vi "2006_FireAtSpecificTimeOnSpecificWeekdays.vi"(8 "error in (no error)":errorcluster) -> (0 "error out":errorcluster)   [LabVIEW 2013]
uses:
  source/Cron.Jenkins/Cron.Jenkins.lvclass/Cron.Jenkins.ctl
  source/Cron.Jenkins/Write Job Name.vi
  <vilib>/addons/_JKI Toolkits/Caraya/classes/Assert/Assert True.vi
  source/Cron/Create Cron Expression.vi
  source/Cron/Compute Next Cron.vi
  source/Cron.Jenkins/Cron.Jenkins.lvclass
  <vilib>/addons/_JKI Toolkits/Caraya/classes/Test/Test.lvclass
  <vilib>/addons/_JKI Toolkits/Caraya/classes/Assert/Assert.lvclass
  source/openCron.lvlib
panel:
  out "after weekend":timestamp
  out "Occurences":timestamp[](array[timestamp])
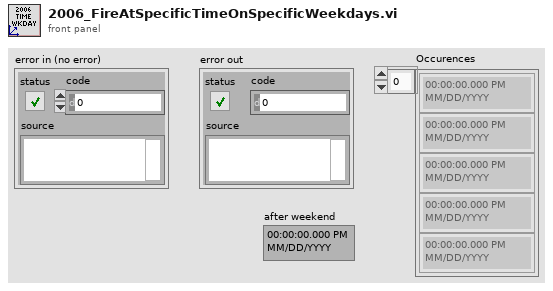
[diagram p1: front panel]
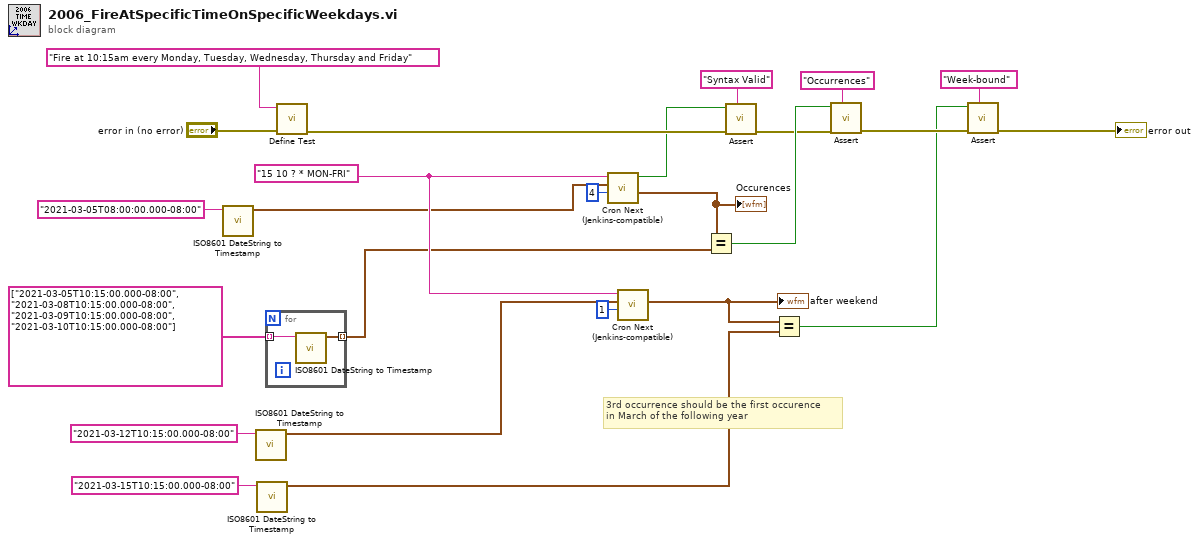
[diagram p0: block diagram]
diagram:
  w12 = "15 10 ? * MON-FRI" ("Expression")
  # "3rd occurrence should be the first occurence\nin March of the following year"
  n1 = call <vilib>:"ISO8601 DateString to Timestamp.vi"("ISO8601 Date String"="2021-03-05T08:00:00.000-08:00" ("Expression")) -> ("Timestamp"=w5:timestamp)  [unwired: 8 in, 2 out]
  n2 = call <vilib>:"ISO8601 DateString to Timestamp.vi"("ISO8601 Date String"="2021-03-12T10:15:00.000-08:00" ("Expression")) -> ("Timestamp"=w2:timestamp)  [unwired: 8 in, 2 out]
  n3 = call <vilib>:"ISO8601 DateString to Timestamp.vi"("ISO8601 Date String"="2021-03-15T10:15:00.000-08:00" ("Expression")) -> ("Timestamp"=w1:timestamp)  [unwired: 8 in, 2 out]
  n4 = for {
    tunnel: string[] ["2021-03-05T10:15:00.000-08:00", "2021-03-08T10:15:00.000-08:00", "2021-03-09T10:15:00.000-08:00", "2021-03-10T10:15:00.000-08:00"] -> [w27] mode=indexing
    tunnel: [w26] -> w3 mode=indexing
    n5 = call <vilib>:"ISO8601 DateString to Timestamp.vi"("ISO8601 Date String"=w27) -> ("Timestamp"=w26:timestamp)  [unwired: 8 in, 2 out]
  }
  n6 = call <vilib>:"Define Test.vi"("error in (no error)"="error in (no error)", "Label (VI Title)"="Fire at 10:15am every Monday, Tuesday, Wednesday, Thursday and Friday") -> ("error out"=w23:errorcluster)  [unwired: 8 in, 1 out]
  n7 = call "Cron Next (Jenkins-compatible).vi"("Nb Occurences (min: 1)"=u16 4, "Reference timestamp (Now)"=w5, "Cron Expression"=w12) -> ("Occurences"=w19:timestamp[], "syntax valid?"=w20:bool)  [unwired: 6 in, 1 out]
  "Occurences" <- w19
  n8 = call "Cron Next (Jenkins-compatible).vi"("Nb Occurences (min: 1)"=u16 1, "Reference timestamp (Now)"=w2, "Cron Expression"=w12) -> ("Next Occurence"=w9:timestamp)  [unwired: 6 in, 2 out]
  "after weekend" <- w9
  n9 = Equal?(x=w19, y=w3) -> (x = y?=w22:bool)
  n10 = call-poly <vilib>:"Assert.vi"("Label"="Syntax Valid" ("Label (VI Title)"), "error in (no error)"=w23, "True?"=w20) -> ("error out"=w21:errorcluster)  [unwired: 7 in, 1 out]
  n11 = Equal?(x=w9, y=w1) -> (x = y?=w10:bool)
  n12 = call-poly <vilib>:"Assert.vi"("Label"="Occurrences" ("Label (VI Title)"), "error in (no error)"=w21, "True?"=w22) -> ("error out"=w14:errorcluster)  [unwired: 7 in, 1 out]
  n13 = call-poly <vilib>:"Assert.vi"("Label"="Week-bound" ("Label (VI Title)"), "error in (no error)"=w14, "True?"=w10) -> ("error out"=→"error out":errorcluster)  [unwired: 7 in, 1 out]
